vi "thermal_optical_capture_7.vi"() -> ()   [LabVIEW 2025]
panel:
  in  "Stop (F)":bool
  in  "Acquisition Control:\nExposure Time [100, 3E7]":dbl=999.0 caption="Acquisition Control::Exposure Time" min=100.0 max=29999995.0
  in  "Analog Control:\nGain [0, 27]":dbl caption="Analog Control::Gain" min=0.0 max=27.045663671679687
  in  "Analog Control:\nBlack Level [-5, 10]":dbl caption="Analog Control::Black Level" min=-5.0000011920928955 max=10.000002384185791
  in  "Analog Control:\nGamma [0.25, 4.00]":dbl=0.800048828125 caption="Analog Control::Gamma" min=0.25 max=4.0 step=0.05
  out "Optical Preview":T1(plugin-control)
  in  "optical capture interval (s)":dbl
  in  "File Path":string="C:\\Digambar\\Metal_thin_wall\\Optical_images\\Optical_images"
  out "Optical Frame Out":string
  in  "Focus":dbl(slide) scale=0.0..100.0
  out "Thermal Frame Out":string
  in  "Thermal Output Folder":path
  in  "thermal capture interval (s)":dbl
  in  "Flag Button":bool
  in  "Stop & Save":bool
  in  "Record":bool
  # "(1) Run VI"
  # "(2) After thermal camera calibration message (in terminal), press START"
  # "(3) Stop & Save"
  # "THERMAL CONTROLS"
  # "(Enter \"28\")"
  # "Thermal Record"
  # "OPTICAL CONTROLS"
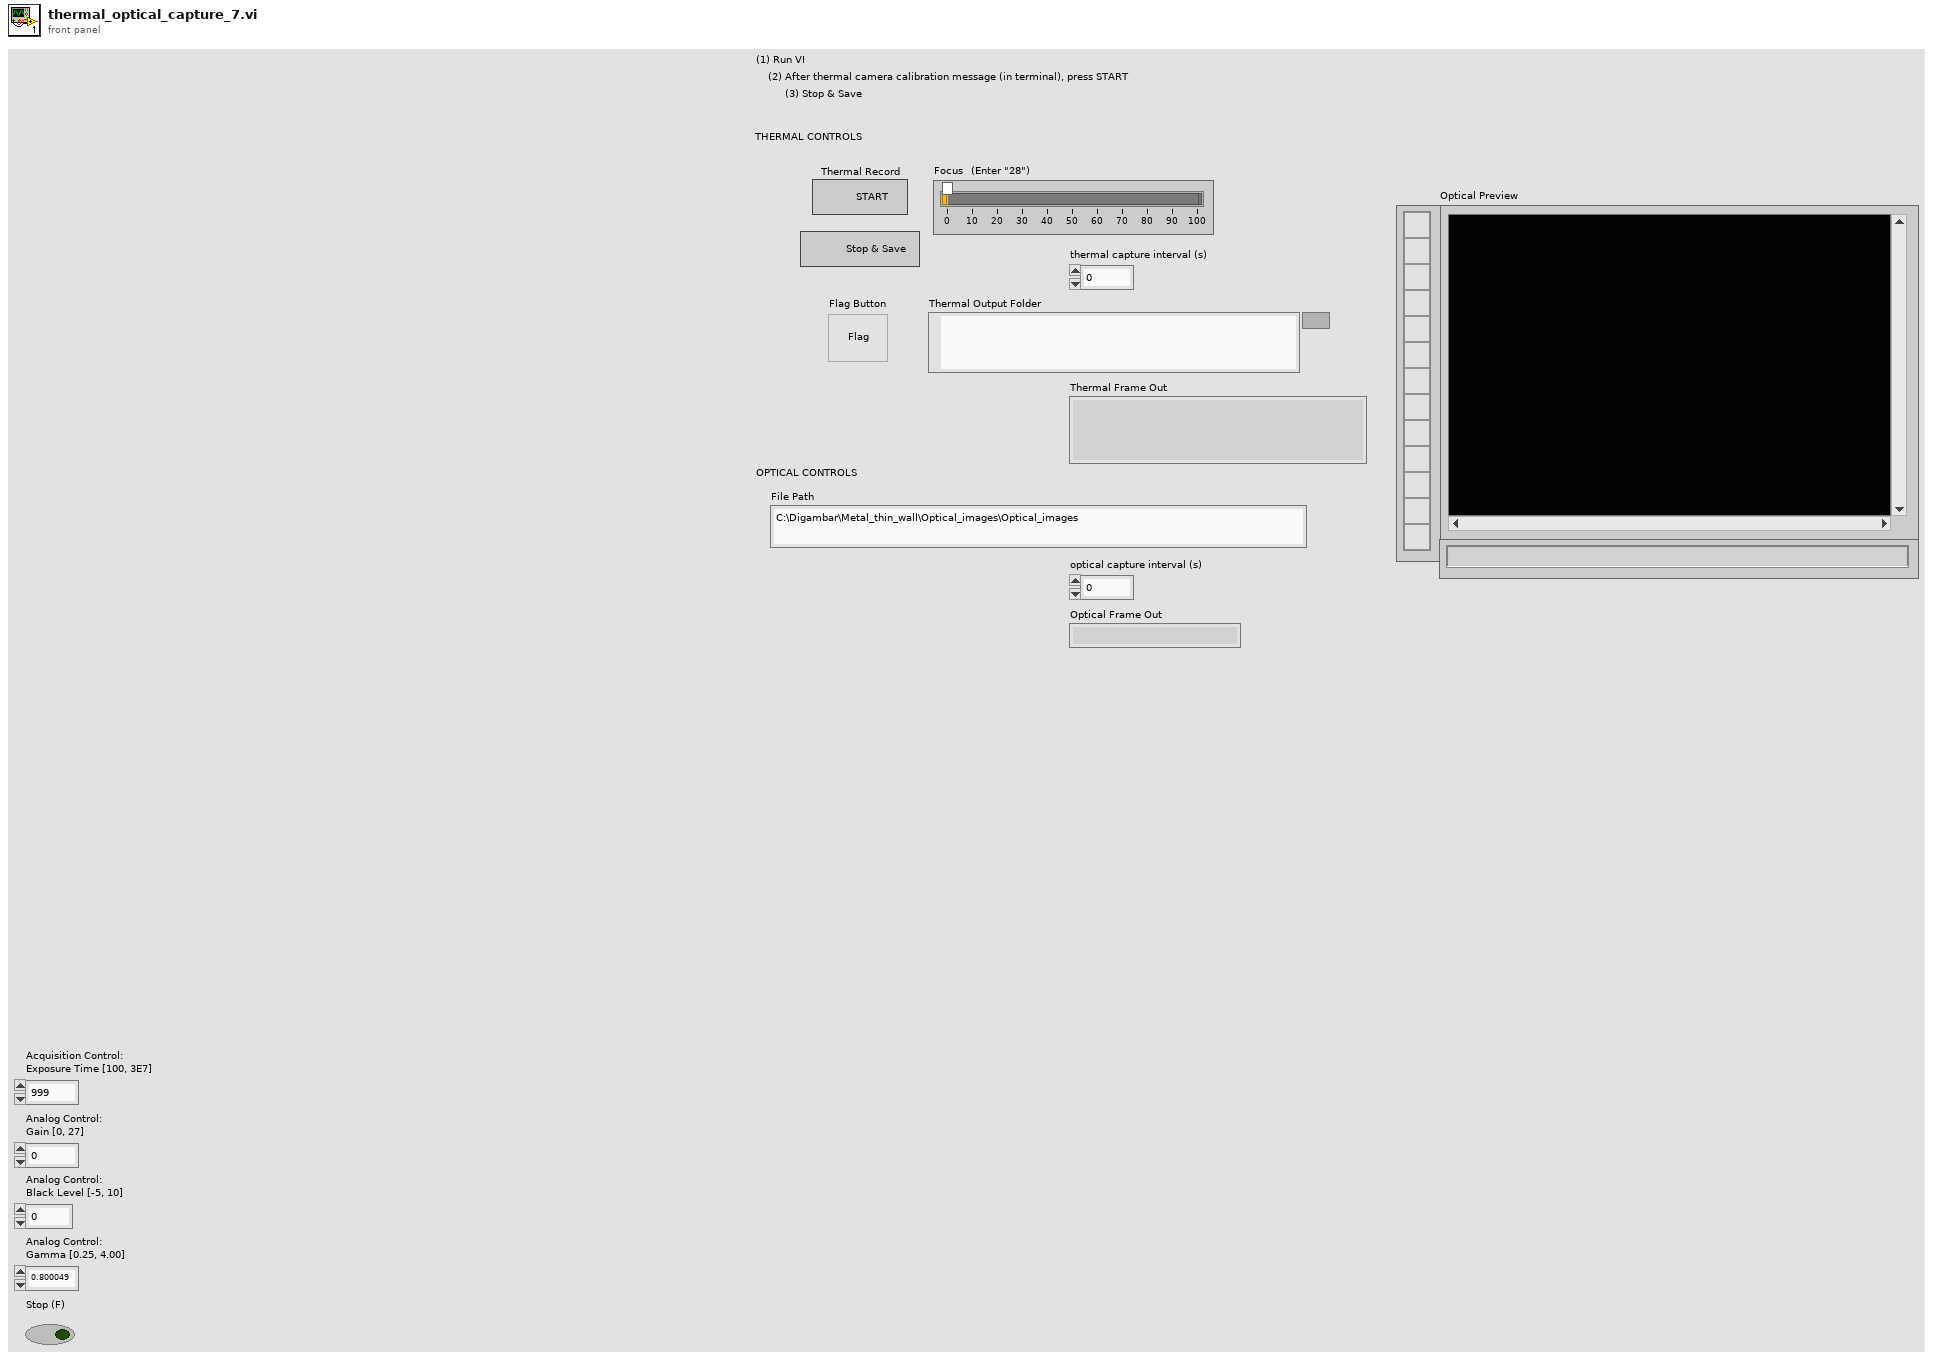
[diagram p1: front panel]
types:
  T1 = typedef "IMAQ Image.ctl" = refnum<image>
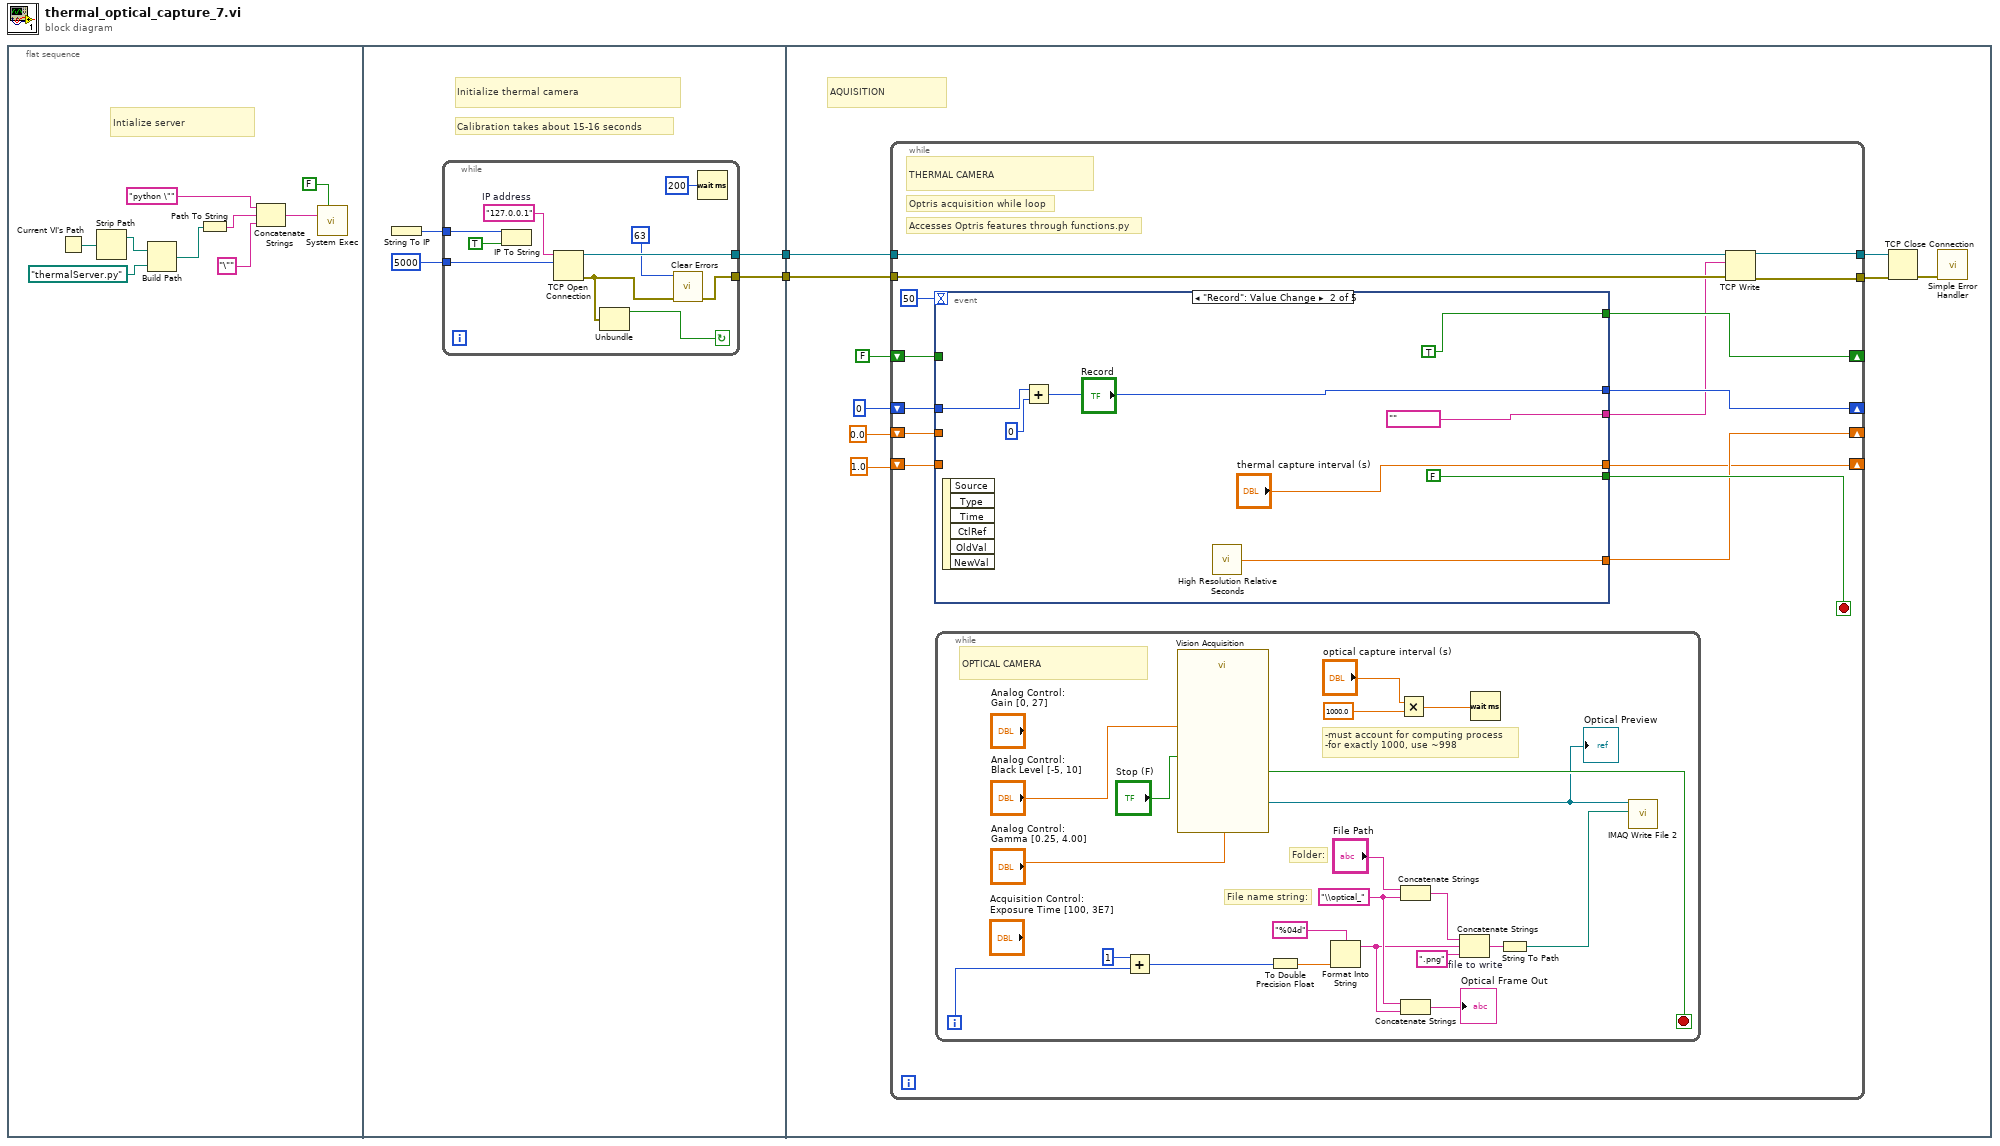
[diagram p0: block diagram]
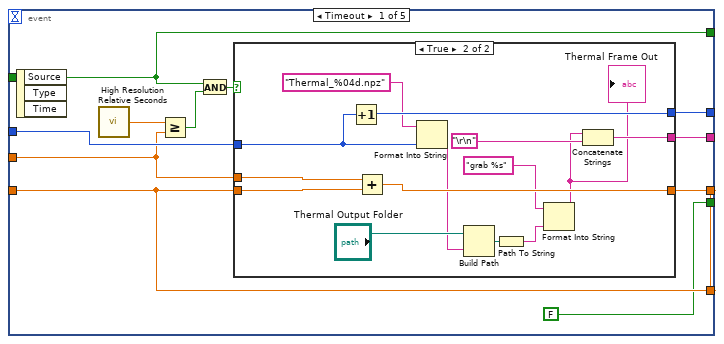
[diagram p2: hidden frame]
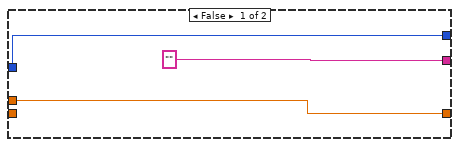
[diagram p3: hidden frame]
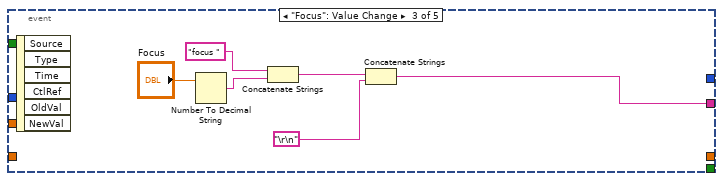
[diagram p4: hidden frame]
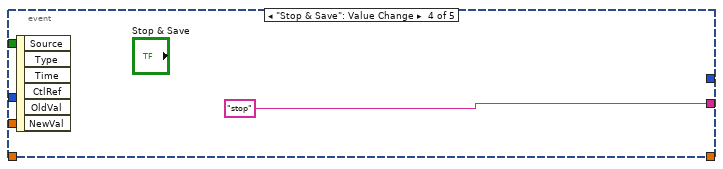
[diagram p5: hidden frame]
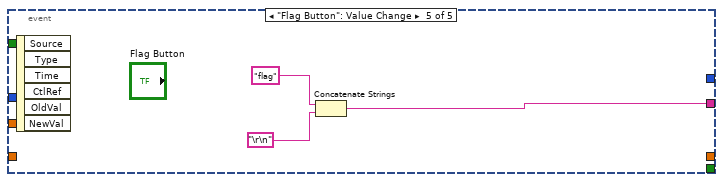
[diagram p6: hidden frame]
diagram:
  n1 = flat-sequence {
    tunnel: [w13] -> w2
    tunnel: [w12] -> w1
    tunnel: w1 -> [w31]
    tunnel: w2 -> [w30]
    frame #0 {
      # "Intialize server"
      n2 = Current VI's Path() -> (path=w6:path)
      n3 = Strip Path(path=w6) -> (stripped path=w7:path)  [unwired: 1 out]
      n4 = Build Path(base path=w7, name or relative path=path "thermalServer.py") -> (appended path=w4:path)
      n5 = Path To String(path=w4) -> (string=w10:string)
      n6 = Concatenate Strings("python \"" ("string"), w10, "\"" ("string")) -> (w9:string)
      n7 = call <vilib>:"System Exec.vi"("wait until completion? (T)"=FALSE, "command line"=w9) -> ()  [unwired: 6 in, 4 out]
    }
    frame #1 {
      # "Initialize thermal camera"
      # "Calibration takes about 15-16 seconds"
      n8 = String To IP() -> (0:w15:u32)  [unwired: 1 in]
      n9 = while {
        tunnel: [w20] -> w13
        tunnel: [w25] -> w12
        tunnel: w15 -> [w24]
        tunnel: u16 5000 ("remote port or service name") -> [w22]
        stop <- w17 continue-if-true
        w16 = "127.0.0.1"  # IP address
        n10 = IP To String(1:TRUE ("dot notation? (F)"), 2:w24) -> ()  [unwired: 1 out]
        n11 = TCP Open Connection(address=w16, remote port or service name=w22) -> (connection ID=w25:refnum<k5>, error out=w21:errorcluster)  [unwired: 3 in]
        n12 = Unbundle(w21) -> ("status"=w17:bool)  [unwired: 2 out]
        n13 = call <vilib>:"Clear Errors.vi"("error in (no error)"=w21, "specific error code to clear (0: all)"=63) -> ("error out"=w20:errorcluster)  [unwired: 4 in, 1 out]
        n14 = Wait (ms)(milliseconds to wait=u32 200) -> ()  [unwired: 1 out]
      }
    }
    frame #2 {
      # "AQUISITION"
      n15 = while {
        tunnel: [w49] -> w32
        tunnel: [w48] -> w33
        tunnel: w31 -> [w46]
        tunnel: w30 -> [w45]
        shift-right: [w43] -> _
        shift-left: u32 0 -> [w44]
        shift-right: [w42] -> _
        shift-left: 0.0 -> [w38]
        shift-right: [w39] -> _
        shift-left: 1.0 -> [w36]
        shift-right: [w40] -> _
        shift-left: FALSE -> [w37]
        stop <- w47 stop-if-true
        # "THERMAL CAMERA"
        # "Optris acquisition while loop"
        # "Accesses Optris features through functions.py"
        n16 = event shown="[1] \"Record\": Value Change" {
          selector: _ -> [_ _ _ _ _]
          dyn-events: _ -> [_ _ _ _ _]
          timeout: 50 -> [_ _ _ _ _]
          tunnel: [w77 "" w107 "stop" w116] -> w35
          tunnel: [FALSE FALSE _ _ _] -> w47
          tunnel: w44 -> [w78 w106 _ _ _]
          tunnel: [w76 w104 _ _ _] -> w43
          tunnel: [w74 w103 _ _ _] -> w42
          tunnel: [w72 TRUE _ _ _] -> w40
          tunnel: [w73 "thermal capture interval (s)" _ _ _] -> w39
          tunnel: w38 -> [w75 _ _ _ _]
          tunnel: w37 -> [w72 _ _ _ _]
          tunnel: w36 -> [w73 _ _ _ _]
          event Timeout {
            n17 = event-data() -> ()  [unwired: 1 in, 3 out]
            n18 = call <vilib>:"High Resolution Relative Seconds.vi"() -> ("relative seconds"=w81:dbl)
            n19 = Greater Or Equal?(x=w81, y=w75) -> (x >= y?=w80:bool)
            n20 = And(x=w72, y=w80) -> (x .and. y?=w79:bool)
            n21 = case shown="True" w79 {
              tunnel: w78 -> [w83 w96]
              tunnel: ["" w97] -> w77
              tunnel: [w83 w95] -> w76
              tunnel: w75 -> [w82 w94]
              tunnel: w73 -> [_ w93]
              tunnel: [w82 w92] -> w74
              frame False {
              }
              frame True {
                n22 = Increment(x=w96) -> (x+1=w95:u32)
                n23 = Add(x=w94, y=w93) -> (x+y=w92:dbl)
                n24 = Format Into String(format string="Thermal_%04d.npz", w96) -> (resulting string=w87:string)  [unwired: 2 in, 1 out]
                n25 = Build Path(base path="Thermal Output Folder", name or relative path=w87) -> (appended path=w89:path)
                n26 = Path To String(path=w89) -> (string=w86:string)
                n27 = Format Into String(format string="grab %s", w86) -> (resulting string=w85:string)  [unwired: 2 in, 1 out]
                "Thermal Frame Out" <- w85
                n28 = Concatenate Strings(w85, "\r\n") -> (w97:string)
              }
            }
          }
          event "Record": Value Change {
            n29 = event-data() -> ()  [unwired: 1 in, 6 out]
            n30 = Add(x=w106, y=u32 0) -> (x+y=w104:u32)
            n31 = call <vilib>:"High Resolution Relative Seconds.vi"() -> ("relative seconds"=w103:dbl)
          }
          event "Focus": Value Change {
            n32 = event-data() -> ()  [unwired: 1 in, 6 out]
            n33 = Number To Decimal String(number="Focus") -> (decimal integer string=w112:string)  [unwired: 1 in]
            n34 = Concatenate Strings("focus ", w112) -> (w109:string)
            n35 = Concatenate Strings(w109, "\r\n") -> (w107:string)
          }
          event "Stop & Save": Value Change {
            n36 = event-data() -> ()  [unwired: 1 in, 6 out]
          }
          event "Flag Button": Value Change {
            n37 = event-data() -> ()  [unwired: 1 in, 6 out]
            n38 = Concatenate Strings("flag", "\r\n") -> (w116:string)
          }
        }
        n39 = while {
          i -> [w51]
          stop <- w69 stop-if-true
          w57 = "\\optical_" ("string")
          # "-must account for computing process\n-for exactly 1000, use ~998"
          # "OPTICAL CAMERA"
          # "Folder:"
          # "File name string:"
          n40 = Add(x=1, y=w51) -> (x+y=w50:i32)
          n41 = call "Vision Acquisition"("Analog Control::Black Level"="Analog Control:\nBlack Level [-5, 10]", "Analog Control::Gamma"="Analog Control:\nGamma [0.25, 4.00]", "Stop (F)"="Stop (F)") -> ("Image Out"=w68:T1, "Stopped"=w69:bool)  [unwired: 22 in, 1 out]
          "Optical Preview" <- w68
          n42 = To Double Precision Float(number=w50) -> (double precision float=w53:dbl)
          n43 = Format Into String(format string="%04d" ("time format string (%c)"), w53) -> (resulting string=w55:string)  [unwired: 2 in, 1 out]
          n44 = Multiply(x="optical capture interval (s)", y=1000.0) -> (x*y=w63:dbl)
          n45 = Concatenate Strings("File Path", w57) -> (w58:string)
          n46 = Concatenate Strings(w57, w55) -> (→"Optical Frame Out":string)
          n47 = Concatenate Strings "file to write"(w58, w55, ".png" ("string")) -> (w65:string)
          n48 = Wait (ms)(milliseconds to wait=w63) -> ()  [unwired: 1 out]
          n49 = String To Path(string=w65) -> (path=w61:path)
          n50 = call-poly "IMAQ Write File 2"("File Path"=w61, "Image"=w68) -> ()  [unwired: 8 in, 2 out]
        }
        n51 = TCP Write(connection ID=w46, data in=w35, error in (no error)=w45) -> (connection ID out=w48:refnum<k5>, error out=w49:errorcluster)  [unwired: 1 in, 1 out]
      }
      n52 = TCP Close Connection(connection ID=w33, error in (no error)=w32) -> (error out=w34:errorcluster)  [unwired: 1 in, 1 out]
      n53 = call <vilib>:"Simple Error Handler.vi"("error in (no error)"=w34) -> ()  [unwired: 4 in, 5 out]
    }
  }
